vi "Move_Ladder.vi"(0 "State":T1={"Tick"=0, "Phase"=0, "PhaseTicks"=0, "Level"=1, "Room"=0, "X10"=0, "Y10"=0, "VY10"=0, "Mode"=0, "Facing"=0, "Run"=0, "Vert"=0, "StandY"=0, "EntryX10"=0, "EntryY10"=0, "EntryMode"=0, "Lives"=4, "Score"=0, "NextLife"=10000, "KeyR"=0, "KeyB"=0, "KeyY"=0, "Torch"=FALSE, "FloorPhase"=0, "Dead"=FALSE, "LevelStart"=FALSE, "Quit"=FALSE, "Sound"=0, "Seed"=12345, "DemoStep"=0, "Tiles"=[], "World"=[], "Enemies"=[], "Highscores"=[], "Name"=[0, 0, 0], "Cursor"=0}, 5 "Jump":bool, 7 "XA10":i32, 11 "error in":errorcluster) -> (4 "Mode":i32, 8 "Y10":i32, 10 "VY10":i32, 15 "error out":errorcluster)   [LabVIEW 2020, in "GH_Engine.lvlib"]
doc: "Claude on a ladder or rope, one tick: climb with Up/Down, stop at the top, on a floor or under a ceiling, fall off the end of a rope, step off sideways, jump off. Inline subVI of Player_Move."
uses:
  GH_Engine.lvlib
  Level/GH_Level.lvlib
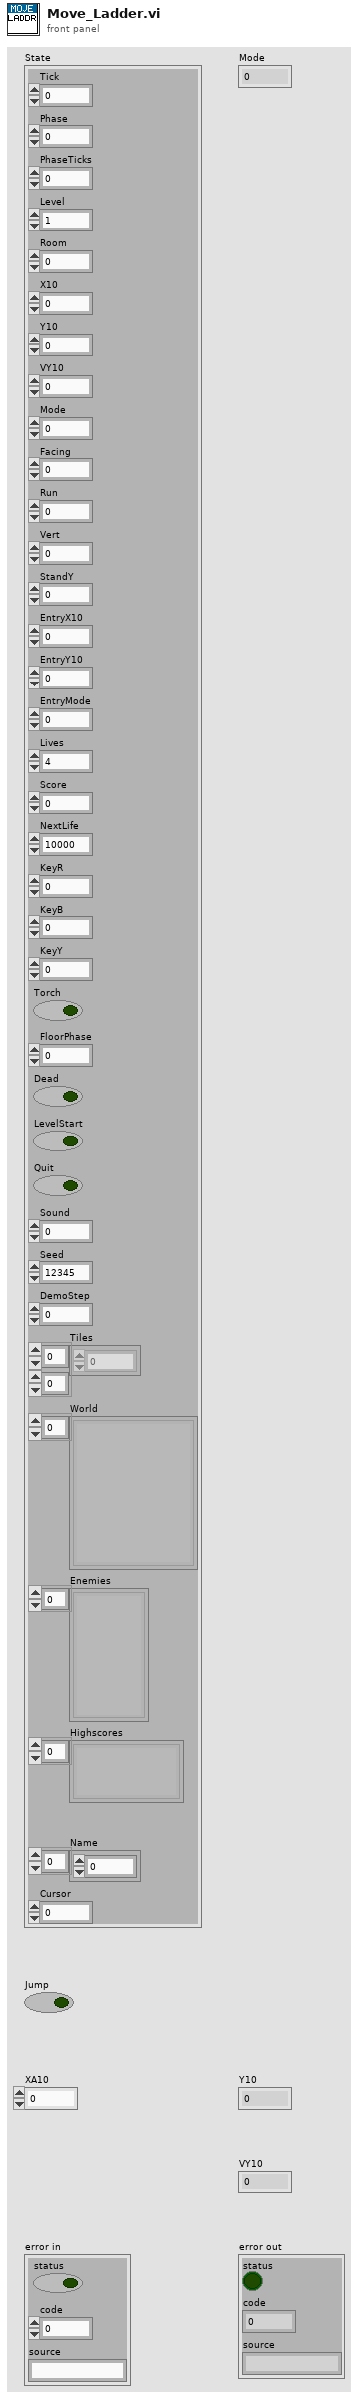
[diagram p1: front panel]
types:
  T1 = cluster{"Tick":u32, "Phase":i32, "PhaseTicks":i32, "Level":i32, "Room":i32, "X10":i32, "Y10":i32, "VY10":i32, "Mode":i32, "Facing":i32, "Run":i32, "Vert":i32, "StandY":i32, "EntryX10":i32, "EntryY10":i32, "EntryMode":i32, "Lives":i32, "Score":i32, "NextLife":i32, "KeyR":i32, "KeyB":i32, "KeyY":i32, "Torch":bool, "FloorPhase":i32, "Dead":bool, "LevelStart":bool, "Quit":bool, "Sound":i32, "Seed":u32, "DemoStep":i32, "Tiles":u8[][], "World":cluster{"ID":string, "Depth":i32, "Column":i32, "Tiles":u8[][]}[], "Enemies":cluster{"Kind":i32, "X10":i32, "Y10":i32, "Dir":i32, "Mode":i32}[], "Highscores":cluster{"Score":i32, "Name":string}[], "Name":i32[], "Cursor":i32}
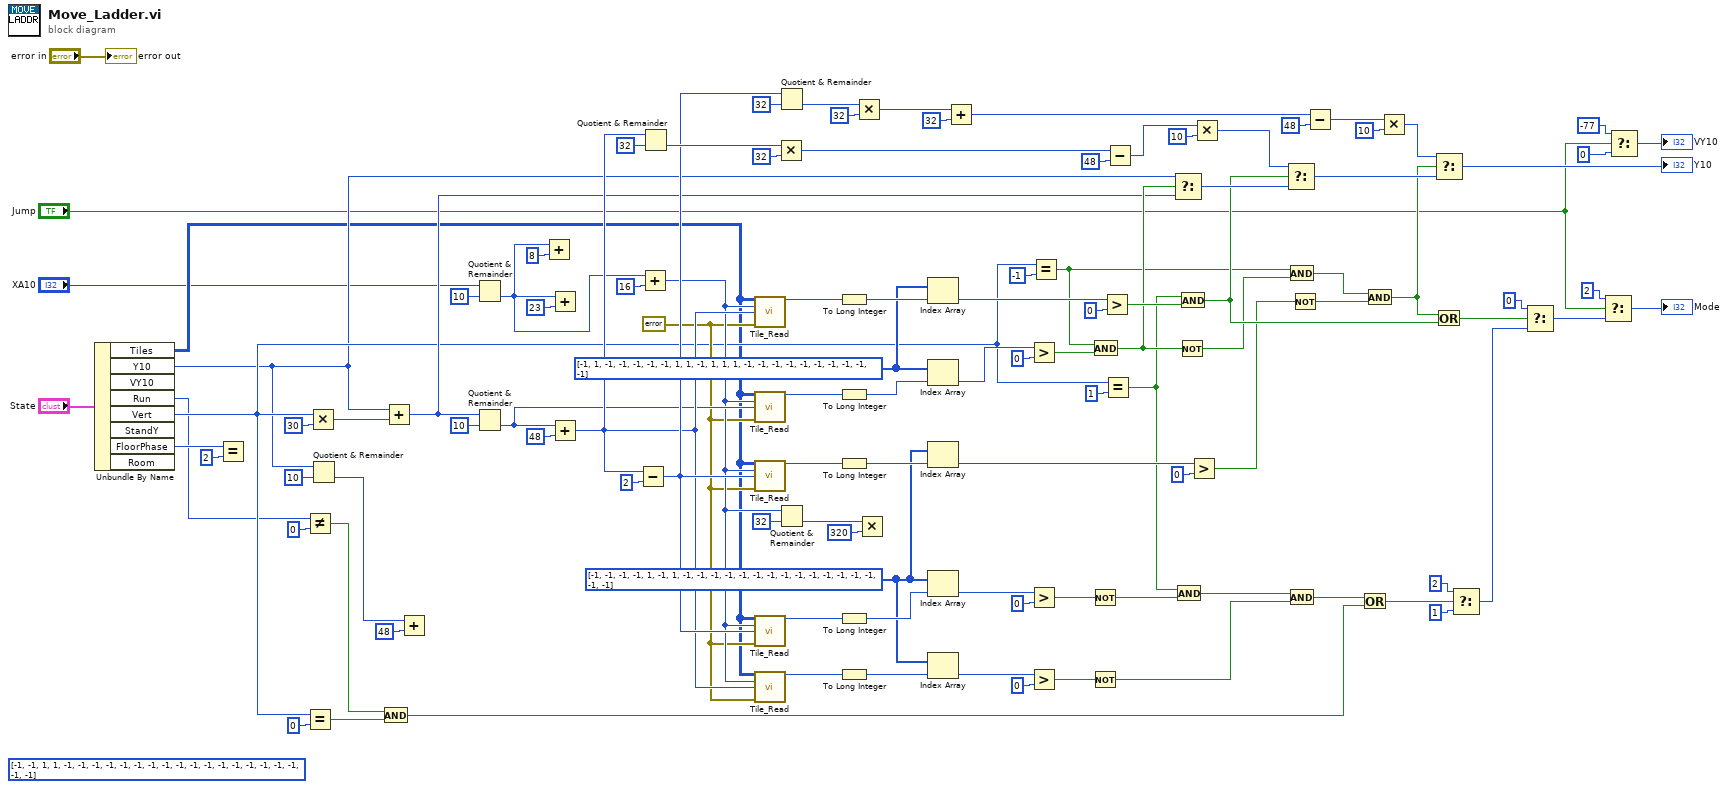
[diagram p0: block diagram]
diagram:
  w13 = errorcluster {"status"=FALSE, "code"=0, "source"=""} ("no error")
  w11 = i32[] [-1, -1, -1, -1, 1, -1, 1, -1, -1, -1, -1, -1, -1, -1, -1, -1, -1, -1, -1, -1, -1, -1, -1] ("Ladder or rope")
  (unwired) i32[] [-1, -1, 1, 1, -1, -1, -1, -1, -1, -1, -1, -1, -1, -1, -1, -1, -1, -1, -1, -1, -1, -1, -1] ("Thin floor")
  w10 = i32[] [-1, 1, -1, -1, -1, -1, -1, 1, 1, -1, 1, 1, 1, -1, -1, -1, -1, -1, -1, -1, -1, -1, -1] ("Solid")
  n1 = Unbundle By Name("State") -> ("Tiles"=w5:u8[][], "Y10"=w6:i32, "Run"=w7:i32, "Vert"=w8:i32, "FloorPhase"=w9:i32)  [unwired: 3 out]
  n2 = Equal?(x=w9, y=2) -> ()  [unwired: 1 out]
  n3 = Not Equal?(x=w7, y=0) -> (x != y?=w89:bool)
  n4 = Equal?(x=w8, y=0) -> (x = y?=w91:bool)
  n5 = Multiply(x=w8, y=30) -> (x*y=w27:i32)
  n6 = Quotient & Remainder(x=w6, y=10) -> (floor(x/y)=w21:i32)  [unwired: 1 out]
  n7 = And(x=w89, y=w91) -> (x .and. y?=w92:bool)
  n8 = Add(x=w6, y=w27) -> (x+y=w28:i32)
  n9 = Add(x=w21, y=48) -> ()  [unwired: 1 out]
  n10 = Quotient & Remainder(x="XA10", y=10) -> (floor(x/y)=w15:i32)  [unwired: 1 out]
  n11 = Quotient & Remainder(x=w28, y=10) -> (floor(x/y)=w30:i32)  [unwired: 1 out]
  n12 = Add(x=w15, y=8) -> ()  [unwired: 1 out]
  n13 = Add(x=w15, y=23) -> ()  [unwired: 1 out]
  n14 = Add(x=w30, y=48) -> (x+y=w32:i32)
  n15 = Subtract(x=w32, y=2) -> (x-y=w44:i32)
  n16 = Add(x=w15, y=16) -> (x+y=w17:i32)
  n17 = Quotient & Remainder(x=w32, y=32) -> (floor(x/y)=w69:i32)  [unwired: 1 out]
  n18 = call "Tile_Read.vi"("Tiles"=w5, "X"=w17, "Y"=w32, "error in"=w13) -> ("Tile"=w62:u8)  [unwired: 10 in, 1 out]
  n19 = call "Tile_Read.vi"("Tiles"=w5, "X"=w17, "Y"=w30, "error in"=w13) -> ("Tile"=w37:u8)  [unwired: 10 in, 1 out]
  n20 = call "Tile_Read.vi"("Tiles"=w5, "X"=w17, "Y"=w44, "error in"=w13) -> ("Tile"=w46:u8)  [unwired: 10 in, 1 out]
  n21 = call "Tile_Read.vi"("Tiles"=w5, "X"=w17, "Y"=w44, "error in"=w13) -> ("Tile"=w74:u8)  [unwired: 10 in, 1 out]
  n22 = call "Tile_Read.vi"("Tiles"=w5, "X"=w17, "Y"=w32, "error in"=w13) -> ("Tile"=w80:u8)  [unwired: 10 in, 1 out]
  n23 = Multiply(x=w69, y=32) -> (x*y=w71:i32)
  n24 = Quotient & Remainder(x=w44, y=32) -> (floor(x/y)=w55:i32)  [unwired: 1 out]
  n25 = Quotient & Remainder(x=w17, y=32) -> (floor(x/y)=w24:i32)  [unwired: 1 out]
  n26 = To Long Integer(number=w62) -> (32bit integer=w63:i32)
  n27 = To Long Integer(number=w37) -> (32bit integer=w38:i32)
  n28 = To Long Integer(number=w46) -> (32bit integer=w47:i32)
  n29 = To Long Integer(number=w74) -> (32bit integer=w75:i32)
  n30 = To Long Integer(number=w80) -> (32bit integer=w81:i32)
  n31 = Multiply(x=w55, y=32) -> (x*y=w57:i32)
  n32 = Multiply(x=w24, y=320) -> ()  [unwired: 1 out]
  n33 = Index Array(array=w10, index=w63) -> (element=w64:i32)
  n34 = Index Array(array=w10, index=w38) -> (element=w39:i32)
  n35 = Index Array(array=w11, index=w47) -> (element=w48:i32)
  n36 = Index Array(array=w11, index=w75) -> (element=w76:i32)
  n37 = Index Array(array=w11, index=w81) -> (element=w82:i32)
  n38 = Add(x=w57, y=32) -> (x+y=w59:i32)
  n39 = Greater?(x=w39, y=0) -> (0:w41:bool)
  n40 = Greater?(x=w76, y=0) -> (0:w78:bool)
  n41 = Greater?(x=w82, y=0) -> (0:w84:bool)
  n42 = Equal?(x=w8, y=-1) -> (x = y?=w34:bool)
  n43 = Not(x=w78) -> (.not. x?=w79:bool)
  n44 = Not(x=w84) -> (.not. x?=w85:bool)
  n45 = And(x=w34, y=w41) -> (x .and. y?=w42:bool)
  n46 = Greater?(x=w64, y=0) -> (0:w66:bool)
  n47 = Equal?(x=w8, y=1) -> (x = y?=w36:bool)
  n48 = Subtract(x=w71, y=48) -> (x-y=w73:i32)
  n49 = Select(t=w6, s=w42, f=w28) -> (s? t:f=w106:i32)
  n50 = And(x=w36, y=w79) -> (x .and. y?=w86:bool)
  n51 = Not(x=w42) -> (.not. x?=w45:bool)
  n52 = And(x=w36, y=w66) -> (x .and. y?=w67:bool)
  n53 = Greater?(x=w48, y=0) -> (0:w50:bool)
  n54 = Multiply(x=w73, y=10) -> (x*y=w105:i32)
  n55 = Select(t=w105, s=w67, f=w106) -> (s? t:f=w107:i32)
  n56 = And(x=w34, y=w45) -> (x .and. y?=w52:bool)
  n57 = And(x=w86, y=w85) -> (x .and. y?=w87:bool)
  n58 = Not(x=w50) -> (.not. x?=w51:bool)
  n59 = Subtract(x=w59, y=48) -> (x-y=w61:i32)
  n60 = Or(x=w87, y=w92) -> (x .or. y?=w96:bool)
  n61 = And(x=w52, y=w51) -> (x .and. y?=w53:bool)
  n62 = Multiply(x=w61, y=10) -> (x*y=w103:i32)
  n63 = Select(t=w103, s=w53, f=w107) -> (s? t:f=→"Y10":i32)
  n64 = Or(x=w53, y=w67) -> (x .or. y?=w94:bool)
  n65 = Select(t=2, s=w96, f=1) -> (s? t:f=w99:i32)
  n66 = Select(t=0, s=w94, f=w99) -> (s? t:f=w100:i32)
  n67 = Select(t=2, s="Jump", f=w100) -> (s? t:f=→"Mode":i32)
  n68 = Select(t=-77, s="Jump", f=0) -> (s? t:f=→"VY10":i32)
  "error out" <- "error in"
